vi "RemoteVI Handle Text Message.vi"(0 "text":string, 1 "acked":u32, 2 "tracking":bool, 3 "seq":u32, 4 "panel":T3, 5 "error in":errorcluster, 6 "popups":T1, 7 "windows":T2(array[cluster]), 8 "mods":u8, 9 "key window":u64, 10 "mods set":u8, 12 "popup since":u32, 20 "view only?":bool) -> (11 "mods set out":u8, 13 "key window out":u64, 14 "acked out":u32, 15 "tracking out":bool, 16 "clicked?":bool, 17 "popups out":T1, 18 "mods out":u8, 19 "error out":errorcluster)   [LabVIEW 2020, in "RemoteVI.lvlib"]
doc: "Handles one text message of a client (docs\\protocol.md section 5) after RemoteVI Parse Input.vi: an ack raises acked to max(acked, seq of the ack) when that seq is not ahead of the client's seq; a mouse or key message goes to the window RemoteVI Route Input.vi picks (the front-most listed window under the pointer, for keys the front-most modal window, else the window last clicked, else the panel; docs\\protocol.md section 7) and is posted to LabVIEW (RemoteVI Post Client Input.vi); x id presses the close box of a listed closable window - WM_SYSCOMMAND SC_CLOSE (RemoteVI Close Window.vi); s id pos stores a splitter move for the server loop (RemoteVI Splitter Request.vi, applied by RemoteVI Apply Splitter.vi when no popup or modal window is open); anything else (invalid) is ignored; with view only? TRUE everything but acks is ignored. No VI Server call."
uses:
  RemoteVI.lvlib
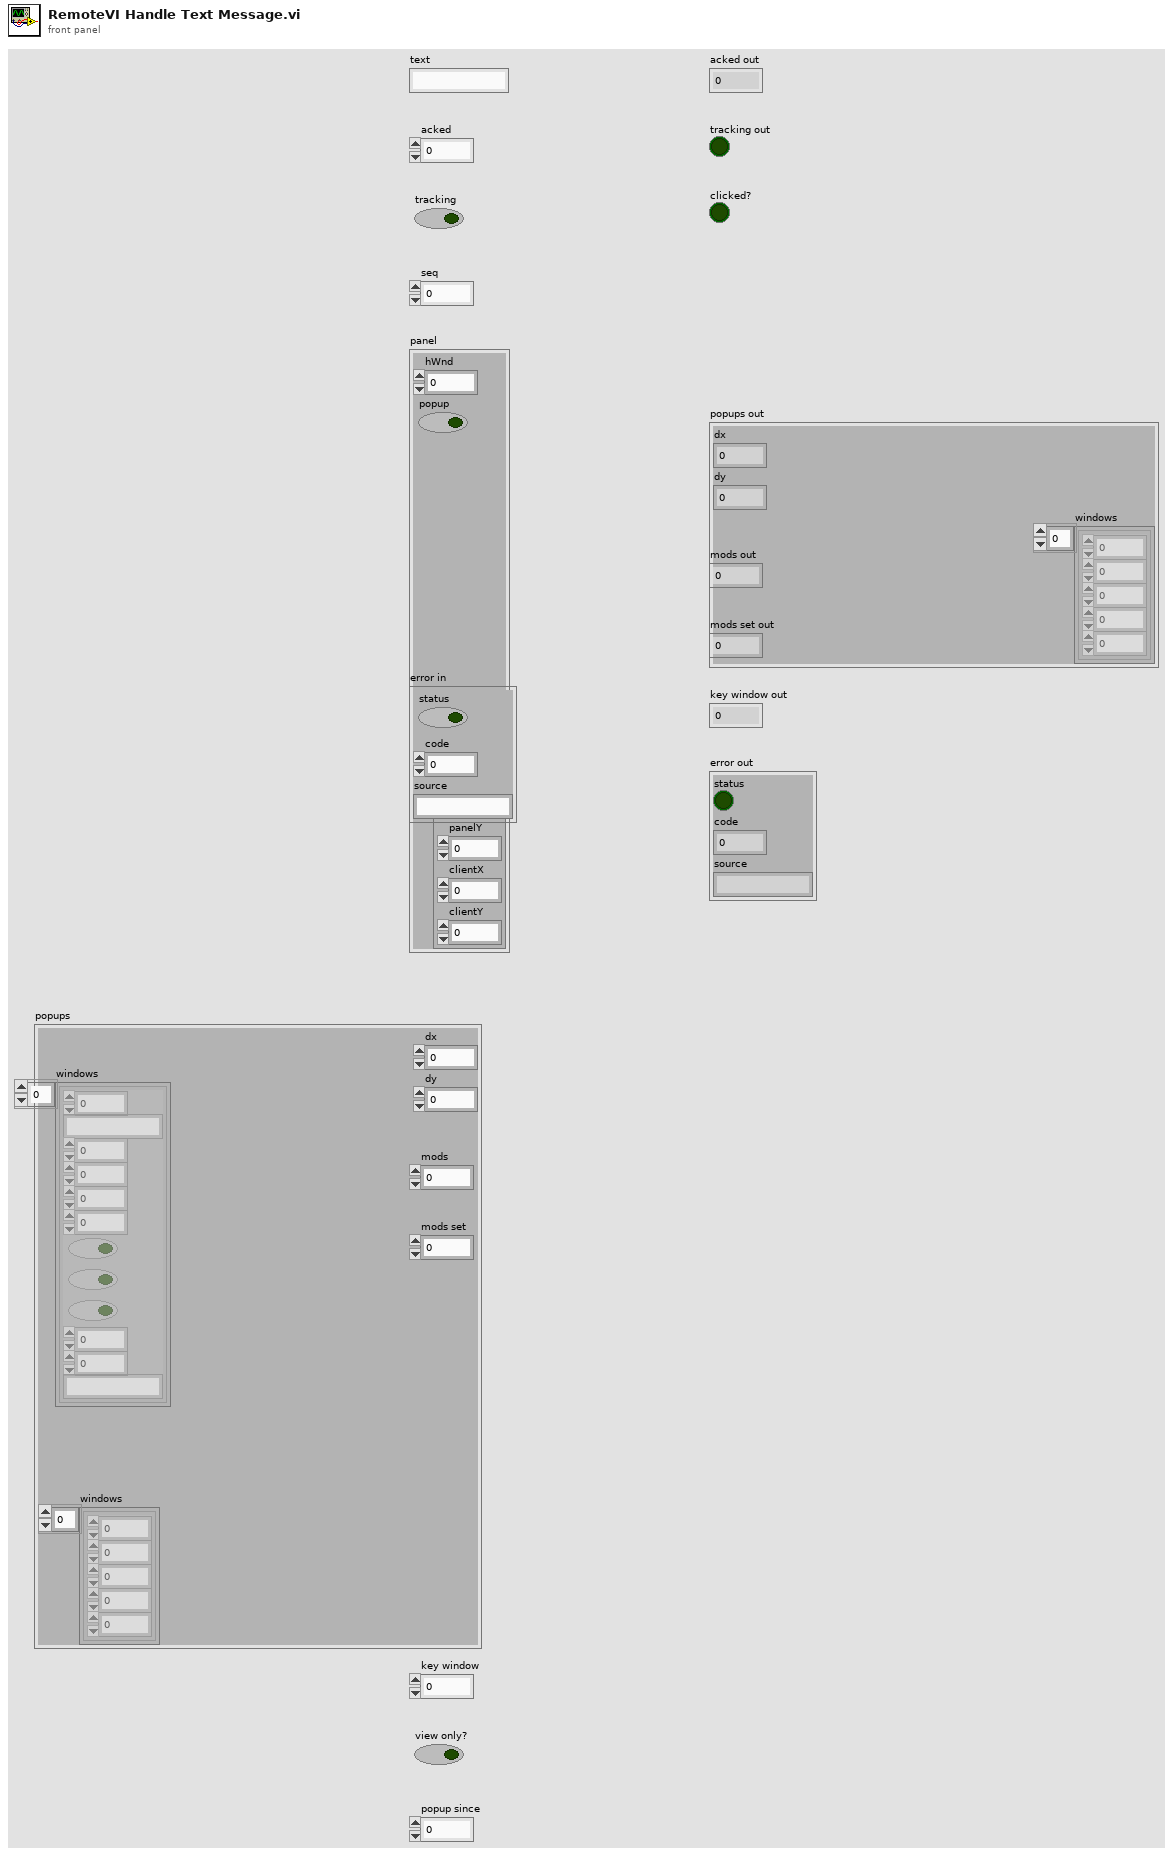
[diagram p1: front panel]
types:
  T1 = cluster{"windows":cluster{"hwnd":u64, "x":i32, "y":i32, "w":i32, "h":i32}[], "dx":i32, "dy":i32}
  T2 = cluster{"id":u64, "title":string, "x":i32, "y":i32, "w":i32, "h":i32, "modal":bool, "active":bool, "closable":bool, "sx":i32, "sy":i32, "class":string}[]
  T3 = cluster{"hWnd":u64, "popup":bool, "geo":cluster{"panelX":i32, "panelY":i32, "clientX":i32, "clientY":i32}}
  T4 = enum16{"invalid", "mouse", "key", "ack", "close", "splitter"}
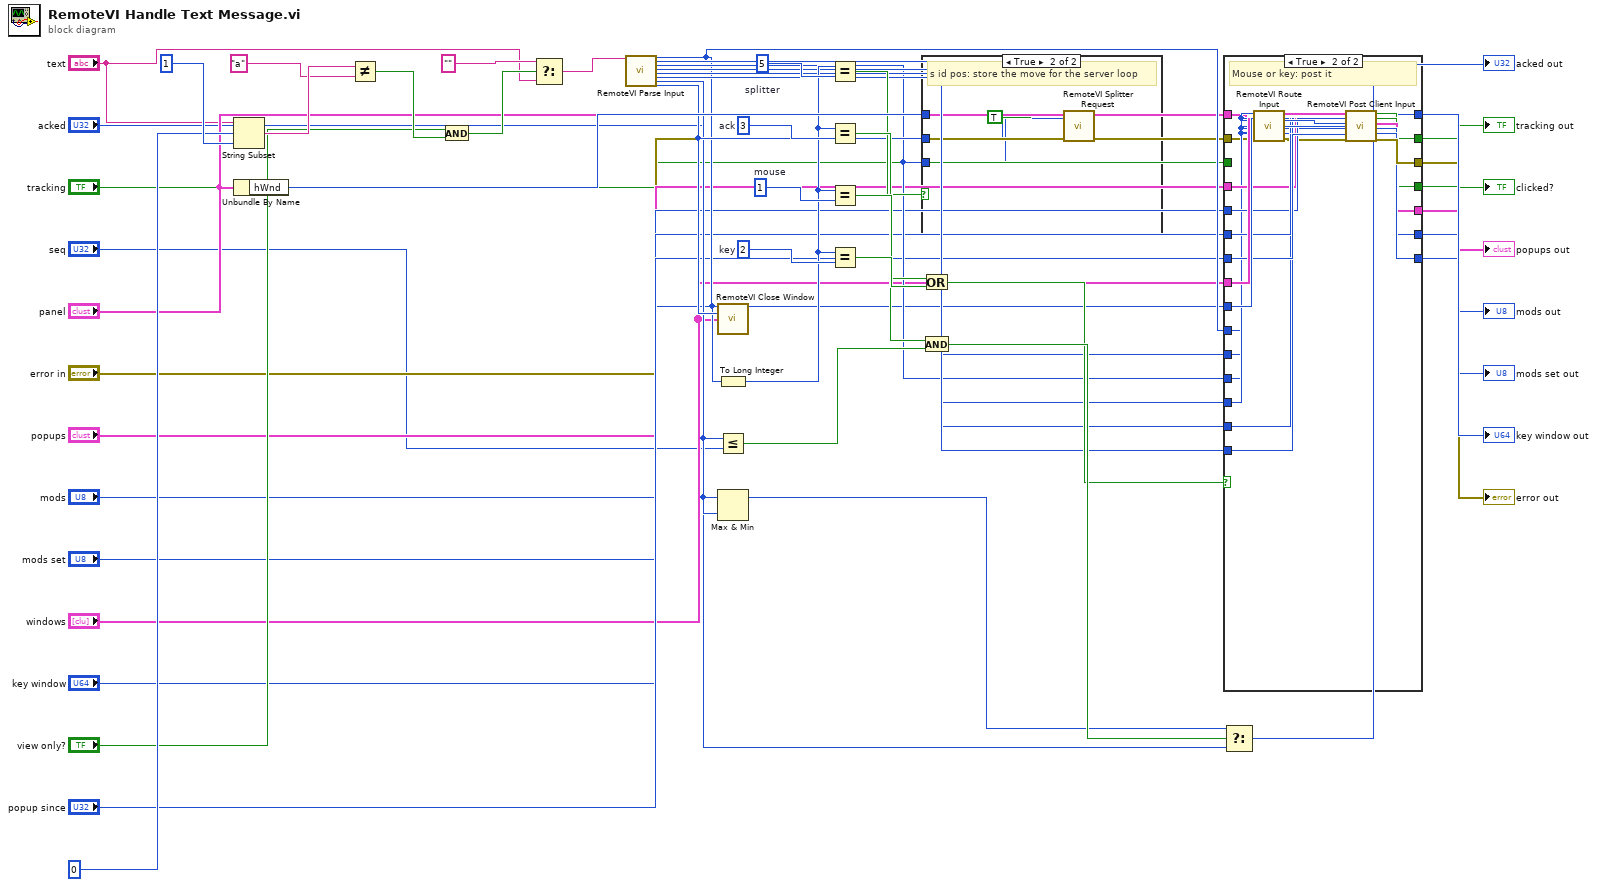
[diagram p0: block diagram]
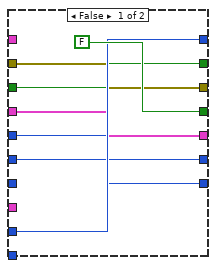
[diagram p2: hidden frame]
diagram:
  w36 = 2  # key
  w35 = 1  # mouse
  w34 = 3  # ack
  w31 = 5  # splitter
  n1 = String Subset(string="text", offset (0)=0, length (rest)=1) -> (substring=w18:string)
  n2 = Unbundle By Name("panel") -> ("hWnd"=w33:u64)
  n3 = Not Equal?(x=w18, y="a") -> (x != y?=w19:bool)
  n4 = And(x="view only?", y=w19) -> (x .and. y?=w20:bool)
  n5 = Select(t="", s=w20, f="text") -> (s? t:f=w21:string)
  n6 = call "RemoteVI Parse Input.vi"("text"=w21) -> ("kind"=w22:T4, "msg"=w23:u32, "x"=w24:i32, "y"=w25:i32, "wParam"=w26:u64, "lParam"=w27:i64, "seq"=w28:u32, "id"=w29:u64)  [unwired: 19 in]
  n7 = call "RemoteVI Close Window.vi"("kind"=w22, "id"=w29, "windows"="windows") -> ()  [unwired: 11 in, 2 out]
  n8 = To Long Integer(number=w22) -> (32bit integer=w30:i32)
  n9 = Less Or Equal?(x=w28, y="seq") -> (x <= y?=w41:bool)
  n10 = Max & Min(x="acked", y=w28) -> (max(x,y)=w42:u32)  [unwired: 1 out]
  n11 = Equal?(x=w30, y=w31) -> (x = y?=w32:bool)
  n12 = Equal?(x=w30, y=w34) -> (x = y?=w37:bool)
  n13 = Equal?(x=w30, y=w35) -> (x = y?=w38:bool)
  n14 = Equal?(x=w30, y=w36) -> (x = y?=w39:bool)
  n15 = case shown="True" w32 {
    tunnel: w33 -> [_ w52]
    tunnel: w29 -> [_ w53]
    tunnel: w24 -> [_ w54]
    frame False {
    }
    frame True {
      # "s id pos: store the move for the server loop"
      n16 = call "RemoteVI Splitter Request.vi"("put?"=TRUE, "hWnd"=w52, "id"=w53, "pos"=w54) -> ()  [unwired: 9 in, 3 out]
    }
  }
  n17 = Or(x=w38, y=w39) -> (x .or. y?=w40:bool)
  n18 = And(x=w37, y=w41) -> (x .and. y?=w43:bool)
  n19 = case shown="True" w40 {
    tunnel: "panel" -> [_ w63]
    tunnel: "error in" -> [w56 w64]
    tunnel: "tracking" -> [w57 _]
    tunnel: "popups" -> [w58 w71]
    tunnel: "mods" -> [w59 w72]
    tunnel: "mods set" -> [w60 w73]
    tunnel: "popup since" -> [_ w74]
    tunnel: "windows" -> [_ w75]
    tunnel: "key window" -> [w61 w76]
    tunnel: w22 -> [_ w65]
    tunnel: w23 -> [_ w66]
    tunnel: w24 -> [_ w67]
    tunnel: w25 -> [_ w68]
    tunnel: w26 -> [_ w69]
    tunnel: w27 -> [_ w70]
    tunnel: [w61 w79] -> w51
    tunnel: [w57 w80] -> w45
    tunnel: [w56 w85] -> w46
    tunnel: [FALSE w81] -> w47
    tunnel: [w58 w82] -> w48
    tunnel: [w59 w83] -> w49
    tunnel: [w60 w84] -> w50
    frame False {
    }
    frame True {
      # "Mouse or key: post it"
      n20 = call "RemoteVI Route Input.vi"("kind"=w65, "panel"=w63, "windows"=w75, "key window"=w76, "msg"=w66, "x"=w67, "y"=w68) -> ("panel out"=w77:T3, "msg out"=w78:u32, "key window out"=w79:u64)  [unwired: 5 in, 1 out]
      n21 = call "RemoteVI Post Client Input.vi"("panel"=w77, "kind"=w65, "msg"=w78, "x"=w67, "y"=w68, "error in"=w64, "wParam"=w69, "mods set"=w73, "lParam"=w70, "popup since"=w74, "popups"=w71, "mods"=w72) -> ("tracking out"=w80:bool, "clicked?"=w81:bool, "popups out"=w82:T1, "mods out"=w83:u8, "mods set out"=w84:u8, "error out"=w85:errorcluster)  [unwired: 2 in]
    }
  }
  "tracking out" <- w45
  "clicked?" <- w47
  "popups out" <- w48
  "mods out" <- w49
  "mods set out" <- w50
  "key window out" <- w51
  "error out" <- w46
  n22 = Select(t=w42, s=w43, f="acked") -> (s? t:f=→"acked out":u32)
